vi "Load Layout By Name.vi"(8 "error in (no error)":errorcluster, 10 "key":string, 11 "Cluster":T7) -> (0 "error out":errorcluster)   [LabVIEW 2020, in "MDI ViewManager.lvlib"]
uses:
  MDI ViewManager.lvlib
  Typedef/Layout.ctl
  <vilib>/Utility/miscctls.llb/LVPointTypeDef.ctl
  <vilib>/Utility/miscctls.llb/LVBoundsTypeDef.ctl
  <vilib>/Utility/miscctls.llb/LVPositionTypeDef.ctl
  <vilib>/Utility/miscctls.llb/LVRectTypeDef.ctl
  Typedef/Update View.ctl
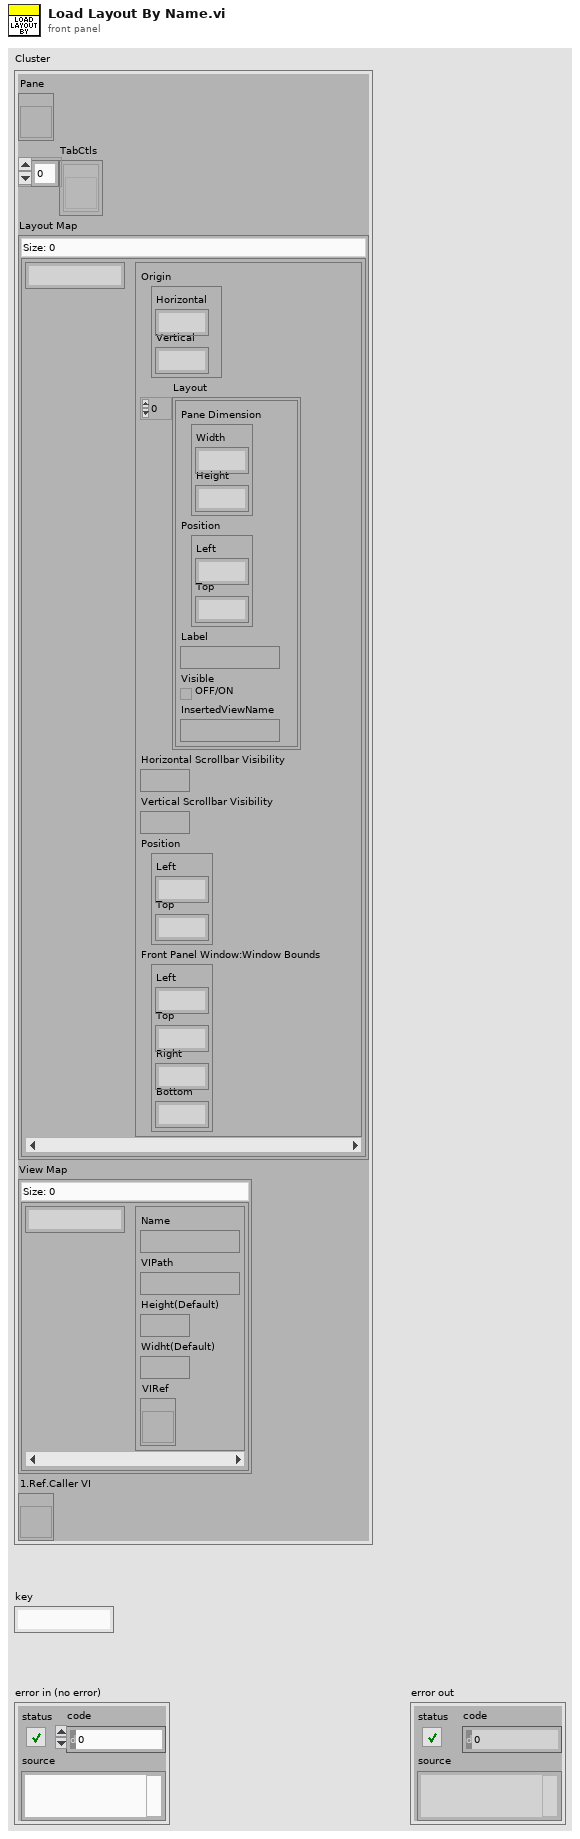
[diagram p1: front panel]
types:
  T1 = typedef "MDI ViewManager.lvlib/Layout.ctl" = cluster{"Origin":T2, "Layout":cluster{"Pane Dimension":T3, "Position":T4, "Label":string, "Visible":bool, "InsertedViewName":string}[], "Horizontal Scrollbar Visibility":enum16{"Always On", "Always Off", "Off While Running"}, "Vertical Scrollbar Visibility":enum16{"Always On", "Always Off", "Off While Running"}, "Position":T4, "Rect":T5}
  T2 = typedef "LVPointTypeDef.ctl" = cluster{"Horizontal":i16, "Vertical":i16}
  T3 = typedef "LVBoundsTypeDef.ctl" = cluster{"Width":u32, "Height":u32}
  T4 = typedef "LVPositionTypeDef.ctl" = cluster{"Left":i32, "Top":i32}
  T5 = typedef "LVRectTypeDef.ctl" = cluster{"Left":i16, "Top":i16, "Right":i16, "Bottom":i16}
  T6 = typedef "MDI ViewManager.lvlib/Update View.ctl" = cluster{"Name":string, "VIPath":path, "Height(Default)":u32, "Widht(Default)":u32, "VIRef":refnum<vi>}
  T7 = cluster{"Pane":refnum<vi>, "TabCtls":refnum<vi>[], "Layout Map":map{string, T1}, "View Map":map{string, T6}, "1.Ref.Caller VI":refnum<vi>}
  T8 = cluster{"Pane Dimension":T3, "Position":T4, "Label":string, "Visible":bool, "InsertedViewName":string}[]
  T9 = enum16{"Always On", "Always Off", "Off While Running"}
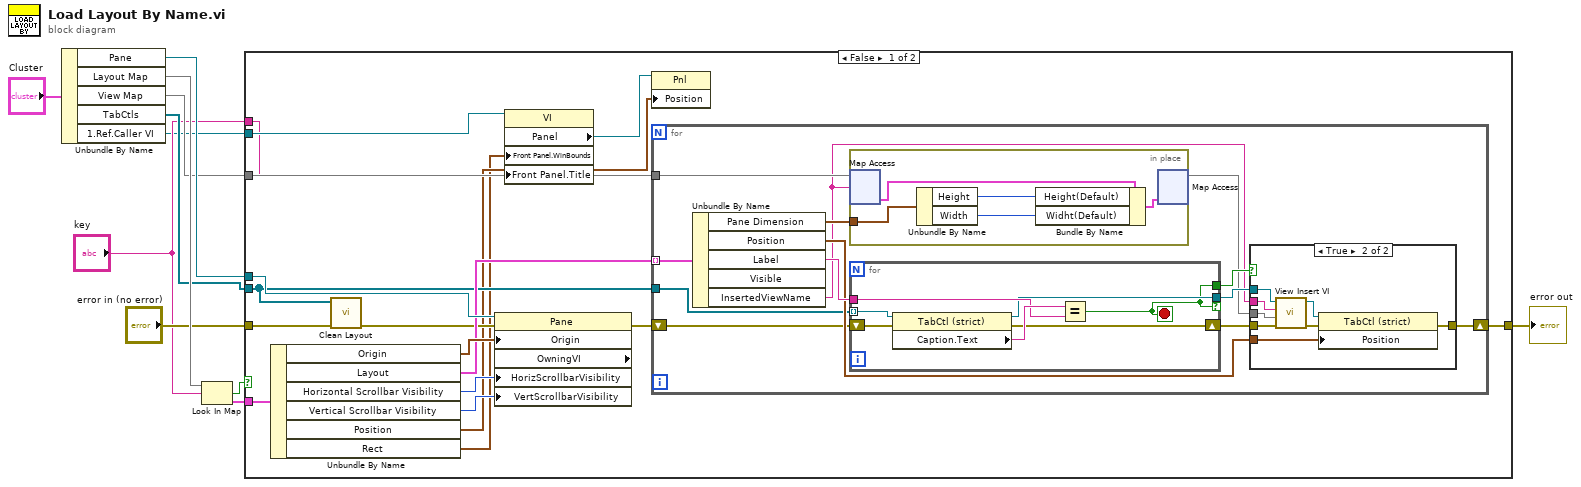
[diagram p0: block diagram]
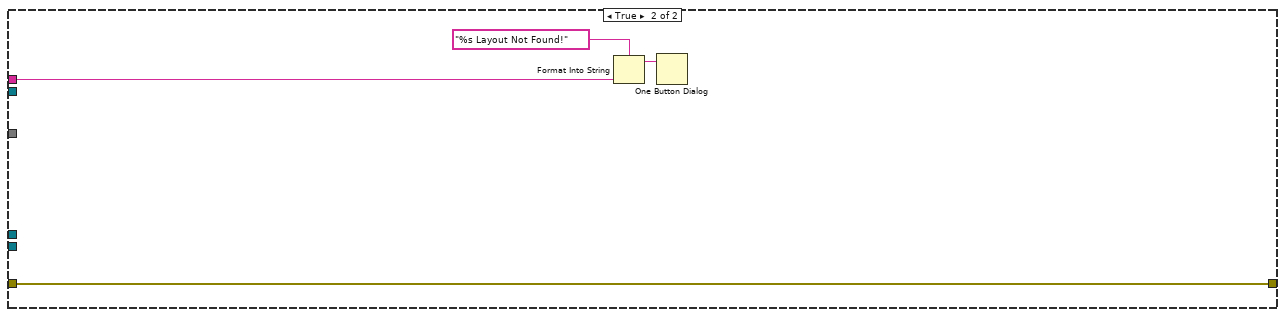
[diagram p3: hidden frame]
diagram:
  n1 = Unbundle By Name("Cluster") -> ("Pane"=w10:refnum<vi>, "Layout Map"=w9:map{string, T1}, "View Map"=w7:map{string, T6}, "TabCtls"=w4:refnum<vi>[], "1.Ref.Caller VI"=w1:refnum<vi>)
  n2 = Look In Map(map=w9, key="key") -> (key not found?=w3:bool, value=w8:T1)  [unwired: 1 in]
  n3 = case shown="False" w3 {
    tunnel: w10 -> [w28 _]
    tunnel: w8 -> [w27 _]
    tunnel: w7 -> [w24 _]
    tunnel: [w22 w66] -> w6
    tunnel: "error in (no error)" -> [w21 w66]
    tunnel: w4 -> [w19 _]
    tunnel: "key" -> [w12 w64]
    tunnel: w1 -> [w13 _]
    frame False {
      n4 = Unbundle By Name(w27) -> ("Origin"=w26:T2, "Layout"=w25:T8, "Horizontal Scrollbar Visibility"=w18:T9, "Vertical Scrollbar Visibility"=w17:T9, "Position"=w15:T4, "Rect"=w14:T5)
      n5 = call "Clean Layout.vi"("error in (no error)"=w21, "TabCtls"=w19) -> ("error out"=w20:errorcluster)  [unwired: 9 in]
      n6 = property class="Pane" props=["Origin", "OwningVI", "HorizScrollbarVisibility", "VertScrollbarVisibility"](reference=w28, error in=w20, "Origin"=w26, "HorizScrollbarVisibility"=w18, "VertScrollbarVisibility"=w17) -> (error out=w23:errorcluster)  [unwired: 2 out]
      n7 = property class="VI"(reference=w13, "Front Panel.WinBounds"=w14, "Front Panel.Title"=w12) -> ("Panel"=w16:refnum<vi>)  [unwired: 1 in, 2 out]
      n8 = property class="Pnl"(reference=w16, "Position"=w15) -> ()  [unwired: 1 in, 2 out]
      n9 = for {
        tunnel: w25 -> [w41] mode=indexing
        tunnel: w19 -> [w29]
        tunnel: w24 -> [w38]
        shift-right: [w34] -> w22
        shift-left: w23 -> [w32]
        n10 = Unbundle By Name(w41) -> ("Pane Dimension"=w36:T3, "Position"=w33:T4, "Label"=w37:string, "InsertedViewName"=w30:string)  [unwired: 1 out]
        n11 = in-place {
          in-place-border: w36 -> [w44]
          n12 = in-place-map #1(w38, w30) -> (w46:T6)  [unwired: 1 in, 1 out]
          n13 = Unbundle By Name(w44) -> ("Height"=w43:u32, "Width"=w42:u32)
          n14 = Bundle By Name(cluster=w46, "Height(Default)"=w43, "Widht(Default)"=w42) -> (w45:T6)
          n15 = in-place-map #1(w45) -> (w35:map{string, T6})  [unwired: 1 in, 2 out]
        }
        n16 = for {
          tunnel: w29 -> [w62] mode=indexing
          tunnel: w37 -> [w60]
          tunnel: [w59] -> w39 if=w56
          tunnel: [w56] -> w40
          shift-right: [w58] -> w31
          shift-left: w32 -> [w57]
          stop <- w56 stop-if-true
          n17 = property class="TabCtl (strict)"(reference=w62, error in=w57) -> (reference out=w59:refnum<vi>, error out=w58:errorcluster, "Caption.Text"=w61:string)
          n18 = Equal?(x=w61, y=w60) -> (x = y?=w56:bool)
        }
        n19 = case shown="True" w40 {
          tunnel: w30 -> [_ w48]
          tunnel: w35 -> [_ w55]
          tunnel: w39 -> [_ w54]
          tunnel: [w47 w50] -> w34
          tunnel: w33 -> [_ w53]
          tunnel: w31 -> [w47 w49]
          frame False {
          }
          frame True {
            n20 = call "View Insert VI.vi"("error in (no error)"=w49, "ViewMap"=w55, "Name"=w48, "TabControl in"=w54) -> ("error out"=w51:errorcluster, "TabControl in 2"=w52:refnum<vi>)  [unwired: 6 in]
            n21 = property class="TabCtl (strict)"(reference=w52, error in=w51, "Position"=w53) -> (error out=w50:errorcluster)  [unwired: 1 out]
          }
        }
      }
    }
    frame True {
      n22 = Format Into String(format string="%s Layout Not Found!" ("message"), w64) -> (resulting string=w63:string)  [unwired: 2 in, 1 out]
      n23 = One Button Dialog(message=w63) -> ()  [unwired: 1 in, 1 out]
    }
  }
  "error out" <- w6
